vi "Prices At.vi"(10 "seconds ago":i32, 11 "price history":dbl[][](array[numeric])) -> (3 "prices":dbl[](array[numeric]))   [LabVIEW 2020, in "Full Featured MCP Server.lvlib"]
doc: "Returns the price of every stock a number of seconds ago (0 = now). A time before the start of the history returns the oldest prices."
uses:
  Full Featured MCP Server.lvlib
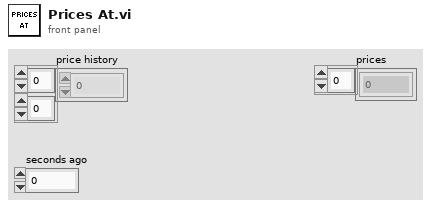
[diagram p1: front panel]
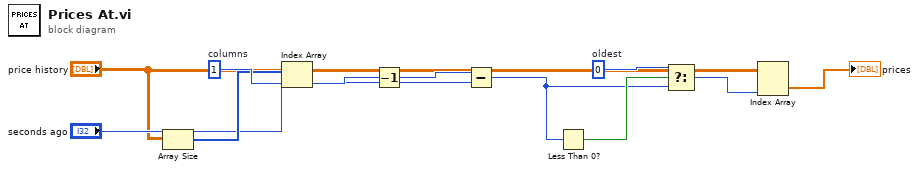
[diagram p0: block diagram]
diagram:
  w9 = 0  # oldest
  w4 = 1  # columns
  n1 = Array Size(array="price history") -> (size(s)=w3:i32[])
  n2 = Index Array(array=w3, index=w4) -> (element=w5:i32)
  n3 = Decrement(x=w5) -> (x-1=w6:i32)
  n4 = Subtract(x=w6, y="seconds ago") -> (x-y=w7:i32)
  n5 = Less Than 0?(x=w7) -> (x < 0?=w8:bool)
  n6 = Select(t=w9, s=w8, f=w7) -> (s? t:f=w10:i32)
  n7 = Index Array(array="price history", index (col)=w10) -> (element=→"prices":dbl[])  [unwired: 1 in]
